vi "SMTP Email [HELO].vi"(4 "error in (no error)":errorcluster caption="entrée d'erreur (pas d'erreur)", 7 "smtp session":T1 caption="session smtp") -> (0 "error out":errorcluster caption="sortie d'erreur", 1 "reply":string caption="réponse", 2 "reply code":i32 caption="code de réponse", 3 "smtp session out":T1 caption="session smtp en sortie")   [LabVIEW 2022 SP3, in "Copie de NI_SMTPEmail.lvlib"]
doc: "Envoie une commande HELO à un serveur SMTP à travers la connexion TCP décrite par \"Session SMTP\" et reçoit la réponse du serveur."
uses:
  Copie de NI_SMTPEmail.lvlib
  SMTP Email Session.ctl
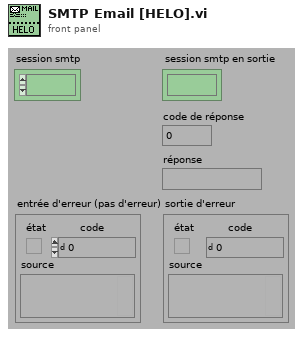
[diagram p1: front panel]
types:
  T1 = typedef "Copie de NI_SMTPEmail.lvlib/SMTP Email Session.ctl" = refnum<k1>
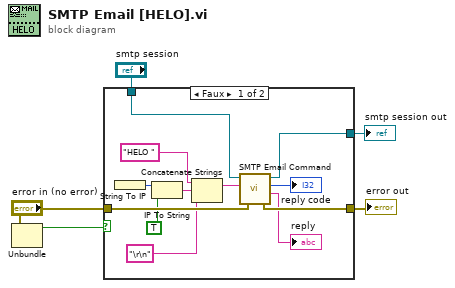
[diagram p0: block diagram]
diagram:
  n1 = Unbundle("error in (no error)") -> ("status"=w1:bool)  [unwired: 2 out]
  n2 = case shown="Faux" w1 {
    tunnel: "smtp session" -> [w15 w19]
    tunnel: [w14 w19] -> w4
    tunnel: [w12 w18] -> w3
    tunnel: "error in (no error)" -> [w11 w18]
    frame False {
      n3 = String To IP() -> (0:w13:u32)  [unwired: 1 in]
      n4 = IP To String(1:TRUE ("dot notation? (F)"), 2:w13) -> (0:w16:string)
      n5 = Concatenate Strings("HELO " ("HELO"), w16, "\r\n" ("HELO")) -> (w8:string)
      n6 = call "SMTP Email Command.vi"("error in (no error)"=w11, "command"=w8, "smtp session"=w15) -> ("error out"=w12:errorcluster, "reply"=→"reply":string, "reply code"=→"reply code":i32, "smtp session out"=w14:T1)  [unwired: 1 in]
    }
    frame True {
    }
  }
  "error out" <- w3
  "smtp session out" <- w4
